vi "Setup.vi"(11 "error in":errorcluster) -> (4 "Application Ref":refnum<vi>, 6 "VI out":refnum<vi>, 15 "error out":errorcluster)   [LabVIEW 2016, in "DronaTest.lvlib"]
uses:
  DronaTest.lvlib
  APIs/Assert/AssertVI/Exec/AssertVIExecRunning.vi
  Drona.lvlib
  APIs/Assert/AssertVI/AssertVI.lvlib
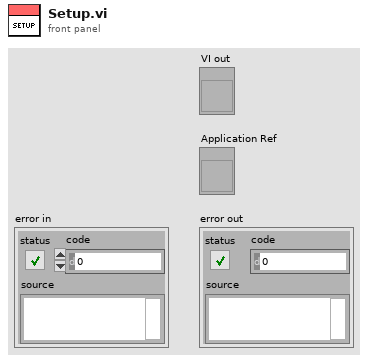
[diagram p1: front panel]
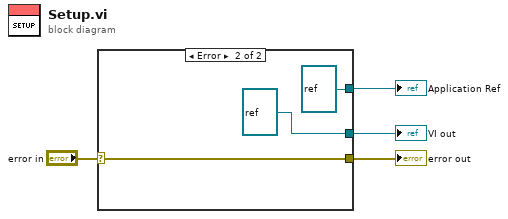
[diagram p0: block diagram]
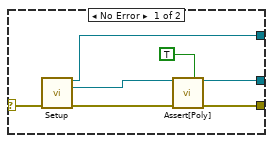
[diagram p2: hidden frame]
diagram:
  n1 = case shown="Error" "error in" {
    selector: "error in" -> [w10 w14]
    tunnel: [w11 refnum<vi> refnum ("Application Ref")] -> w4
    tunnel: [w8 refnum<vi> refnum ("VI Reference Out")] -> w2
    tunnel: [w6 w14] -> w1
    frame No Error {
      n2 = call "Setup.vi"("error in"=w10) -> ("Application Ref"=w11:refnum<vi>, "VI Reference Out"=w9:refnum<vi>, "error out"=w7:errorcluster)  [unwired: 12 in]
      n3 = call-poly "Assert[Poly].vi"("VI Reference In"=w9, "Assert Only? (F)"=TRUE, "Error In"=w7) -> ("VI Reference Out"=w8:refnum<vi>, "Error Out"=w6:errorcluster)  [unwired: 10 in, 1 out]
    }
    frame Error {
    }
  }
  "Application Ref" <- w4
  "VI out" <- w2
  "error out" <- w1
